vi "RemoteVI Classify Client Frame.vi"(0 "complete?":bool, 5 "fin":bool, 7 "opcode":u8, 9 "close code":u16) -> (4 "text?":bool, 6 "ping?":bool, 8 "close?":bool, 10 "close code out":u16)   [LabVIEW 2020, in "RemoteVI.lvlib"]
doc: "Decides what to do with a decoded client frame (RemoteVI WS Decode Client Frame.vi, docs\\protocol.md section 4): text? for a complete final text frame; ping? for a complete ping; close? for a complete close frame (answered with 1000), a complete binary, continuation or other unexpected frame (1008 - policy violation) or a protocol violation the decoder reported (its close code). Pure."
uses:
  RemoteVI.lvlib
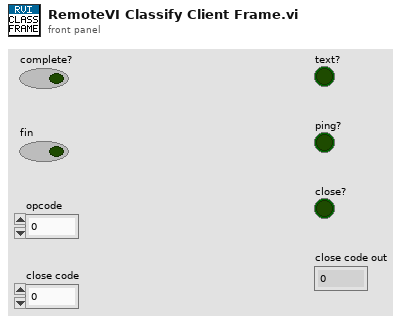
[diagram p1: front panel]
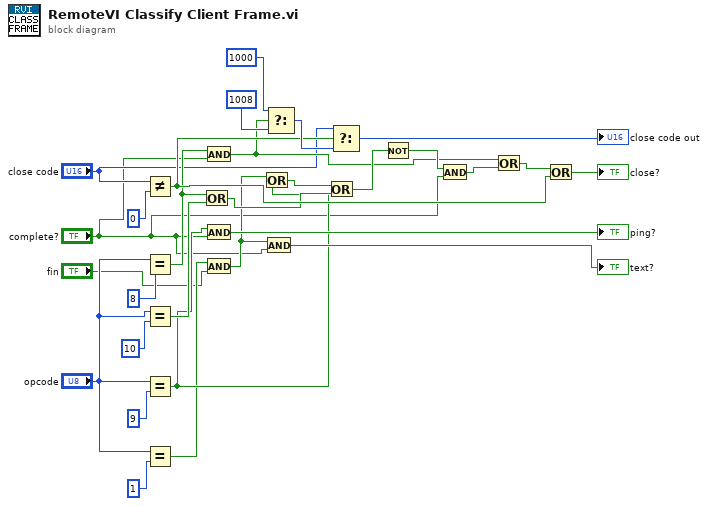
[diagram p0: block diagram]
diagram:
  n1 = Not Equal?(x="close code", y=u16 0) -> (x != y?=w23:bool)
  n2 = Equal?(x="opcode", y=u8 8) -> (x = y?=w10:bool)
  n3 = Equal?(x="opcode", y=u8 10) -> (x = y?=w12:bool)
  n4 = Equal?(x="opcode", y=u8 9) -> (x = y?=w11:bool)
  n5 = Equal?(x="opcode", y=u8 1) -> (x = y?=w9:bool)
  n6 = Or(x=w10, y=w12) -> (x .or. y?=w18:bool)
  n7 = And(x=w10, y="complete?") -> (x .and. y?=w16:bool)
  n8 = And(x=w11, y="complete?") -> (x .and. y?=→"ping?":bool)
  n9 = And(x=w9, y="fin") -> (x .and. y?=w13:bool)
  n10 = Or(x=w13, y=w11) -> (x .or. y?=w17:bool)
  n11 = And(x=w13, y="complete?") -> (x .and. y?=→"text?":bool)
  n12 = Select(t=u16 1000, s=w16, f=u16 1008) -> (s? t:f=w28:u16)
  n13 = Or(x=w17, y=w18) -> (x .or. y?=w19:bool)
  n14 = Select(t="close code", s=w23, f=w28) -> (s? t:f=→"close code out":u16)
  n15 = Not(x=w19) -> (.not. x?=w20:bool)
  n16 = And(x=w20, y="complete?") -> (x .and. y?=w21:bool)
  n17 = Or(x=w16, y=w21) -> (x .or. y?=w24:bool)
  n18 = Or(x=w24, y=w23) -> (x .or. y?=→"close?":bool)
